vi "App Init.vi"(8 "error in (no error)":errorcluster, 10 "Volatus API":refnum<class "VolatusAPI.lvclass">, 11 "DemoApp in":refnum<class "DemoApp.lvclass">) -> (0 "error out":errorcluster, 3 "DemoApp out":refnum<class "DemoApp.lvclass">)   [LabVIEW 2020, in "VolatusDemo.lvlib" / "DemoApp.lvclass"]
uses:
  DemoApp.lvclass
  Volatus/VolatusAPI/VolatusAPI.lvclass
  DemoApp.lvclass/DemoApp.ctl
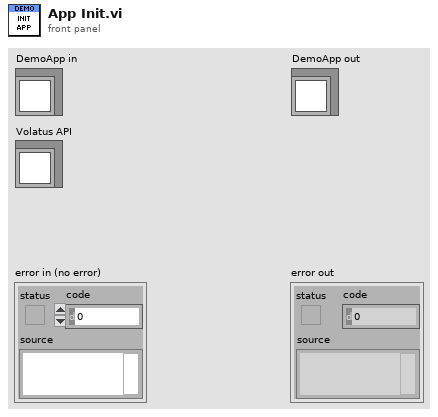
[diagram p1: front panel]
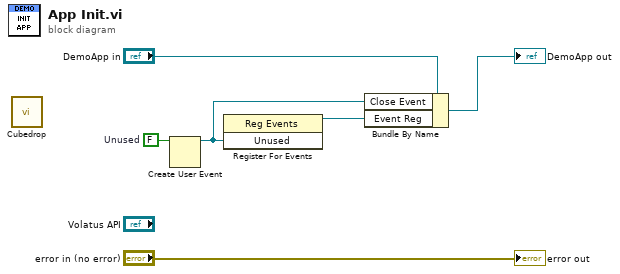
[diagram p0: block diagram]
diagram:
  w5 = FALSE  # Unused
  n1 = call "Cubedrop.vi"() -> ()  [unwired: 12 in]
  n2 = Create User Event(user event datatype=w5) -> (user event=w2:refnum<user-event>)  [unwired: 1 in, 1 out]
  n3 = register-events(w2) -> (reference out=w3:refnum<event-registration>)  [unwired: 2 in, 1 out]
  n4 = Bundle By Name(cluster="DemoApp in", "Close Event"=w2, "Event Reg"=w3) -> (→"DemoApp out":refnum<class "DemoApp.lvclass">)
  "error out" <- "error in (no error)"
